vi "OwnBuild20261013_CreateDLL.vi"() -> ()   [LabVIEW 2024]
uses:
  <vilib>/AppBuilder/AB_API/DLL/NI_AB_API_DLL.lvclass
panel:
  out "error out":errorcluster caption="错误输出"
  in  "Save Project Path":path
  in  "Output Name":string caption="共享库文件名"
  in  "Destination":path
  in  "Spec Name":string caption="程序生成规范名称"
  in  "Member ID":string
  in  "Project Path":path
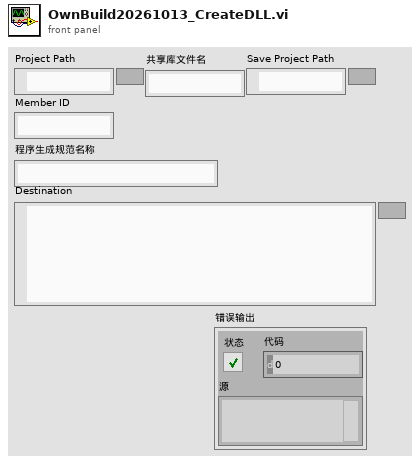
[diagram p1: front panel]
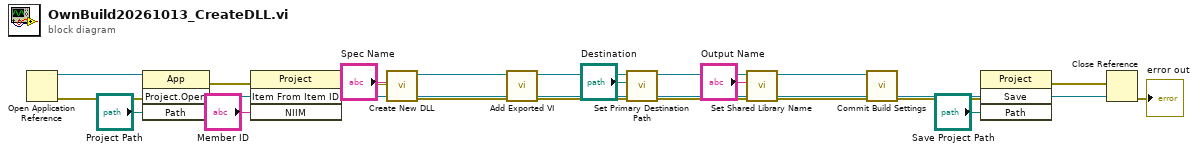
[diagram p0: block diagram]
diagram:
  n1 = Open Application Reference() -> (0:w21:errorcluster, 3:w23:refnum<vi>)  [unwired: 4 in]
  n2 = invoke class="App" method="Project.Open"(reference=w23, error in=w21, "Path"="Project Path") -> (error out=w18:errorcluster, "Project:Open"=w20:refnum<vi>)  [unwired: 1 in, 2 out]
  n3 = invoke class="Project" method="Item From Item ID"(reference=w20, error in=w18, "NIIM"="Member ID") -> (error out=w16:errorcluster, "GetItemFromNIIM"=w14:refnum<vi>)  [unwired: 1 in, 2 out]
  n4 = call <vilib>:"Create New DLL.vi"("error in (no error)"=w16, "Build specification name"="Spec Name", "Project Refnum"=w20) -> ("error out"=w13:errorcluster, "DLL out"=w15:refnum<class "NI_AB_API_DLL.lvclass">)  [unwired: 7 in]
  n5 = call-dynamic "Add Exported VI.vi"("error in (no error)"=w13, "ProjectItem Refnum"=w14, "DLL in"=w15) -> ("error out"=w10:errorcluster, "DLL out"=w12:refnum<class "NI_AB_API_DLL.lvclass">)  [unwired: 7 in]
  n6 = call-dynamic "Set Primary Destination Path.vi"("error in (no error)"=w10, "Destination path"="Destination", "Build in"=w12) -> ("error out"=w7:errorcluster, "Build out"=w9:refnum<class "NI_AB_API_DLL.lvclass">)  [unwired: 7 in]
  n7 = call-dynamic "Set Shared Library Name.vi"("error in (no error)"=w7, "Shared library file name"="Output Name", "DLL in"=w9) -> ("error out"=w5:errorcluster, "DLL out"=w6:refnum<class "NI_AB_API_DLL.lvclass">)  [unwired: 7 in]
  n8 = call-dynamic "Commit Build Settings.vi"("error in (no error)"=w5, "DLL in"=w6) -> ("error out"=w3:errorcluster)  [unwired: 8 in, 1 out]
  n9 = invoke class="Project" method="Save"(reference=w20, error in=w3, "Path"="Save Project Path") -> (error out=w2:errorcluster)  [unwired: 1 in, 3 out]
  n10 = Close Reference(reference=w20, error in (no error)=w2) -> (error out=→"error out":errorcluster)
